vi "UE_TriState_Condition.vi"(1 "condition_met":bool, 2 "sample_valid":bool) -> (0 "state_code":i32)   [LabVIEW 2026]
doc: "INTENT: Evaluate result as -1 UNKNOWN, 0 FALSE or 1 TRUE; invalid sample never passes. INPUTS: sample_valid (bool), condition_met (bool). OUTPUTS: state_code (int32). DESIGN CONSTRAINT: Quality states stale and invalid must be converted to sample_valid=false by Parameter Registry. REQUIREMENTS: SRS-F-022. No physical hardware side effects. Acceptance requires native LabVIEW compilation and behavioral testing."
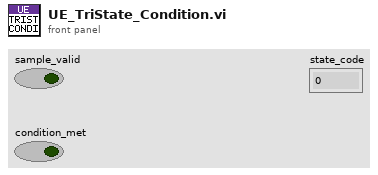
[diagram p1: front panel]
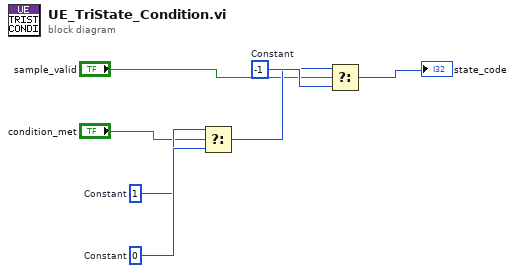
[diagram p0: block diagram]
diagram:
  w6 = -1  # Constant
  w4 = 0  # Constant
  w3 = 1  # Constant
  n1 = Select(t=w3, s="condition_met", f=w4) -> (s? t:f=w5:i32)
  n2 = Select(t=w5, s="sample_valid", f=w6) -> (s? t:f=→"state_code":i32)
